vi "Set Label from Name.vi"(8 "error in":errorcluster, 11 "Element in":refnum<class "Element.lvclass">) -> (0 "error out":errorcluster, 3 "Element out":refnum<class "Element.lvclass">)   [LabVIEW 2026, in "Element.lvclass"]
doc: "Set element label using the elements name."
uses:
  Element.lvclass
  Element.lvclass/Element.ctl
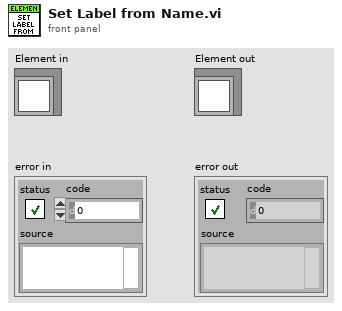
[diagram p1: front panel]
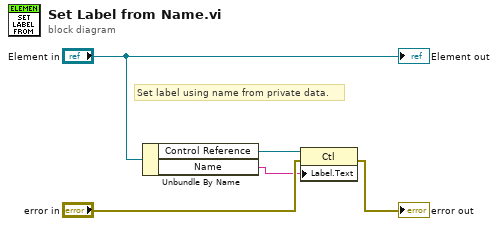
[diagram p0: block diagram]
diagram:
  # "Set label using name from private data."
  n1 = Unbundle By Name("Element in") -> ("Control Reference"=w2:refnum<vi>, "Name"=w1:string)
  n2 = property class="Ctl"(reference=w2, error in="error in", "Label.Text"=w1) -> (error out=→"error out":errorcluster)  [unwired: 1 out]
  "Element out" <- "Element in"
